vi "Display Module - Switch On and Off.vi"(0 "Image Refs":T1[](array[typedef]), 11 "IMAQ Display Refs":refnum<vi>[](array[refnum])) -> ()   [LabVIEW 2021]
uses:
  <vilib>/vision/Image Controls.llb/IMAQ Image.ctl
  <vilib>/Utility/miscctls.llb/LVPointTypeDef.ctl
panel:
  in  "Quit":bool
  # "Click on a display to change its state."
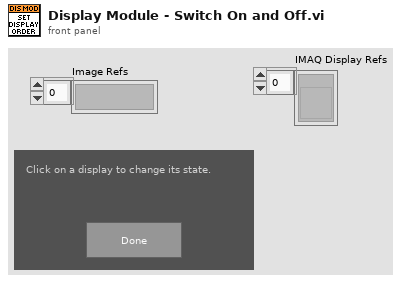
[diagram p1: front panel]
types:
  T1 = typedef "IMAQ Image.ctl" = refnum<image>
  T2 = enum16{"Always On", "Always Off", "Off While Running"}
  T3 = typedef "LVPointTypeDef.ctl" = cluster{"Horizontal":i16, "Vertical":i16}
  T4 = enum16{"User-specified Font", "Application Font", "System Font", "Dialog Font"}
  T5 = cluster{"Desired Font (Application)":enum16{"User-specified Font", "Application Font", "System Font", "Dialog Font"}, "[User-specified Font]":cluster{"Font Name":string, "Size":i16, "Strikeout?":bool, "Italic?":bool, "Underline?":bool, "Outline?":bool, "Shadow?":bool, "Bold?":bool, "Rotation Angle":dbl}, "Horizontal Alignment":i16, "Vertical Alignment":i16}
  T6 = cluster{"Font Name":string, "Size":i16, "Strikeout?":bool, "Italic?":bool, "Underline?":bool, "Outline?":bool, "Shadow?":bool, "Bold?":bool, "Rotation Angle":dbl}
  T7 = typedef "LVRectTypeDef.ctl" = cluster{"Left":i16, "Top":i16, "Right":i16, "Bottom":i16}
  T8 = typedef "LVBoundsTypeDef.ctl" = cluster{"Width":u32, "Height":u32}
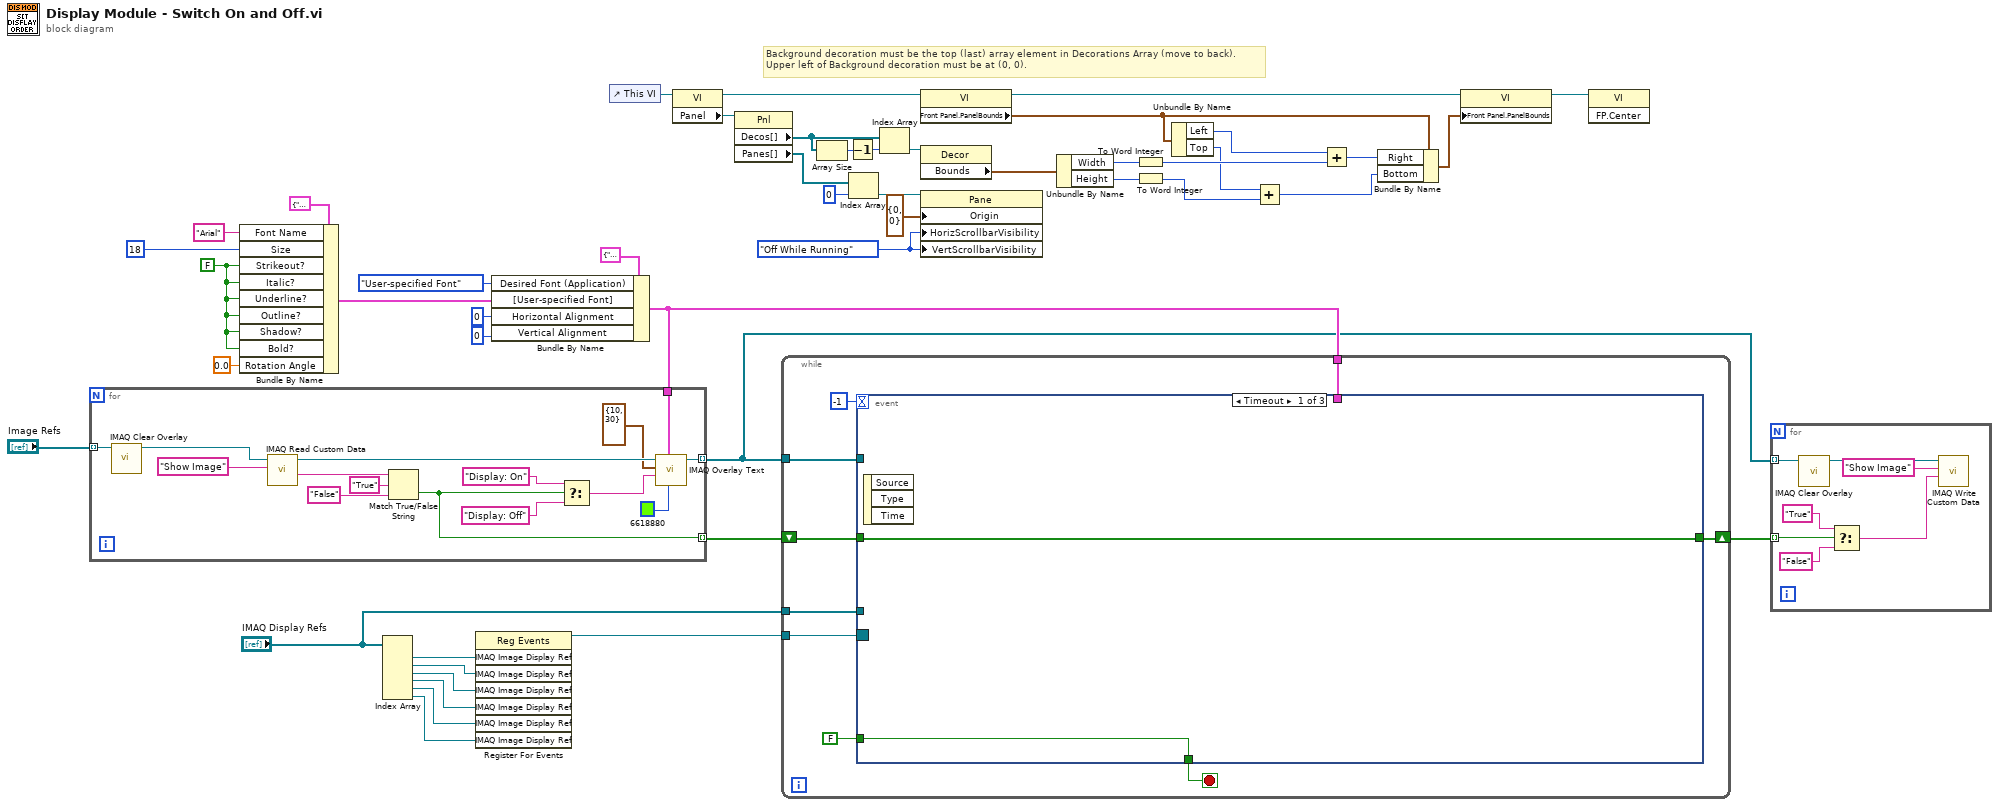
[diagram p0: block diagram]
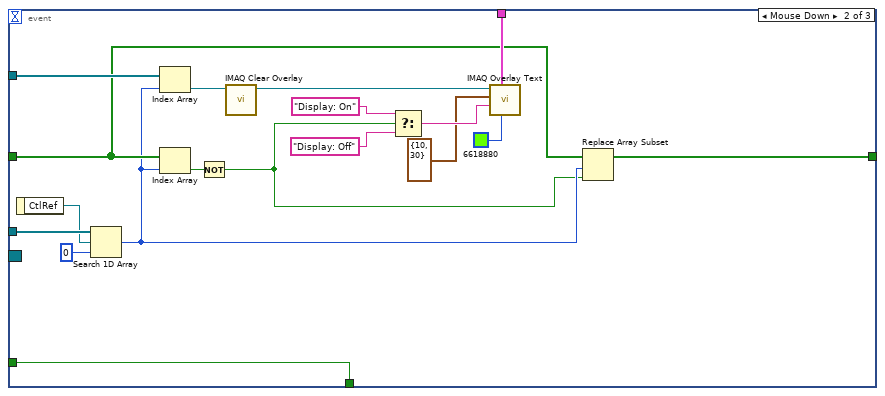
[diagram p2: hidden frame]
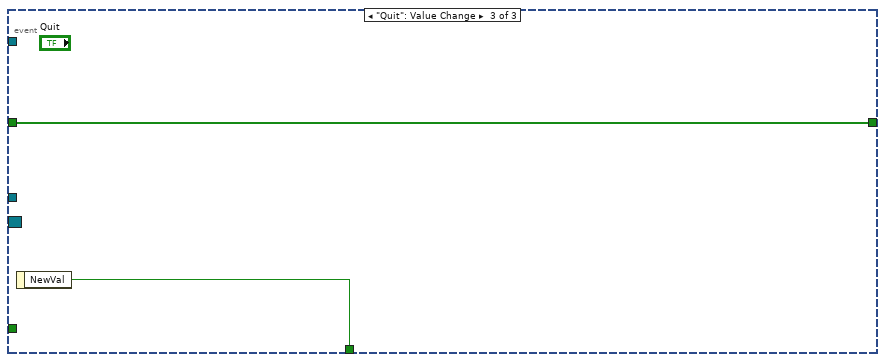
[diagram p3: hidden frame]
diagram:
  w15 = T2."Off While Running" ("Vertical Scrollbar Visibility")
  w38 = FALSE ("Strikeout?")
  # "Background decoration must be the top (last) array element in Decorations Array (move to back).\nUpper left of Background decoration must be at (0, 0)."
  n1 = Bundle By Name(cluster=T6 {"Font Name"="", "Size"=0, "Strikeout?"=FALSE, "Italic?"=FALSE, "Underline?"=FALSE, "Outline?"=FALSE, "Shadow?"=FALSE, "Bold?"=FALSE, "Rotation Angle"=0.0} ("[User-specified Font]"), "Font Name"="Arial", "Size"=i16 18, "Strikeout?"=w38, "Italic?"=w38, "Underline?"=w38, "Outline?"=w38, "Shadow?"=w38, "Bold?"=w38, "Rotation Angle"=0.0) -> (w40:T6)
  n2 = Index Array(array="IMAQ Display Refs") -> (element #1=w33:refnum<vi>, element #2=w37:refnum<vi>, element #3=w34:refnum<vi>, element #4=w35:refnum<vi>, element #5=w36:refnum<vi>, element #6=w31:refnum<vi>)  [unwired: 6 in]
  n3 = register-events(w33, w37, w34, w35, w36, w31) -> (reference out=w32:refnum<event-registration>)  [unwired: 2 in, 1 out]
  n4 = Bundle By Name(cluster=T5 {"Desired Font (Application)"=enum."Application Font", "[User-specified Font]"={"Font Name"="", "Size"=12, "Strikeout?"=FALSE, "Italic?"=FALSE, "Underline?"=FALSE, "Outline?"=FALSE, "Shadow?"=FALSE, "Bold?"=FALSE, "Rotation Angle"=0.0}, "Horizontal Alignment"=0, "Vertical Alignment"=0} ("Font, Size & Style"), "Desired Font (Application)"=T4."User-specified Font", "[User-specified Font]"=w40, "Horizontal Alignment"=i16 0, "Vertical Alignment"=i16 0) -> (w28:T5)
  n5 = for {
    tunnel: "Image Refs" -> [w52] mode=indexing
    tunnel: w28 -> [w53]
    tunnel: [w50] -> w27 mode=indexing
    tunnel: [w49] -> w30 mode=indexing
    n6 = call "IMAQ Clear Overlay"("Image"=w52) -> ("Image Out"=w51:T1)  [unwired: 9 in, 1 out]
    n7 = call "IMAQ Read Custom Data"("Key"="Show Image", "Image"=w51) -> ("Custom Data Out"=w63:string, "Image (duplicate)"=w59:T1)  [unwired: 7 in, 1 out]
    n8 = Match True/False String(2:"False" ("false string"), 3:"True" ("true string"), 4:w63) -> (0:w49:bool)  [unwired: 1 out]
    n9 = Select(t="Display: On" ("false string"), s=w49, f="Display: Off" ("false string")) -> (s? t:f=w55:string)
    n10 = call "IMAQ Overlay Text"("Text Color (black)"=u32 6618880, "Font, Size & Style"=w53, "String"=w55, "Origin"=cluster{"X":i32, "Y":i32} {"X"=10, "Y"=30}, "Image"=w59) -> ("Image Out"=w50:T1)  [unwired: 5 in, 1 out]
  }
  n11 = control-ref of="This VI"() -> (w8:refnum<vi>)
  n12 = property class="VI"(reference=w8) -> (reference out=w16:refnum<vi>, "Panel"=w9:refnum<vi>)  [unwired: 1 in, 1 out]
  n13 = property class="Pnl"(reference=w9) -> ("Decos[]"=w7:refnum<vi>[], "Panes[]"=w12:refnum<vi>[])  [unwired: 1 in, 2 out]
  n14 = while {
    tunnel: w32 -> [w69]
    shift-right: [w64] -> w26
    shift-left: w30 -> [w67]
    tunnel: "IMAQ Display Refs" -> [w66]
    tunnel: w28 -> [w65]
    tunnel: w27 -> [w68]
    stop <- w72 stop-if-true
    n15 = event shown="[0] Timeout" {
      selector: w69 -> [_ _ _]
      dyn-events: _ -> [_ _ _]
      timeout: -1 -> [_ _ _]
      tunnel: [w73 w92 w94] -> w72
      tunnel: FALSE -> [w73 w92 _]
      tunnel: w68 -> [_ w81 _]
      tunnel: w67 -> [w74 w78 w93]
      tunnel: w66 -> [_ w91 _]
      tunnel: w65 -> [_ w82 _]
      tunnel: [w74 w77 w93] -> w64
      event Timeout {
        n16 = event-data() -> ()  [unwired: 1 in, 3 out]
      }
      event Mouse Down {
        n17 = event-data() -> ("CtlRef"=w90:refnum<vi>)  [unwired: 1 in]
        n18 = Search 1D Array(1D array=w91, element=w90, start index (0)=0) -> (index of element=w76:i32)
        n19 = Index Array(array=w81, index=w76) -> (element=w80:T1)
        n20 = Index Array(array=w78, index=w76) -> (element=w88:bool)
        n21 = Not(x=w88) -> (.not. x?=w75:bool)
        n22 = call "IMAQ Clear Overlay"("Image"=w80) -> ("Image Out"=w79:T1)  [unwired: 9 in, 1 out]
        n23 = Select(t="Display: On" ("false string"), s=w75, f="Display: Off" ("false string")) -> (s? t:f=w84:string)
        n24 = call "IMAQ Overlay Text"("Text Color (black)"=u32 6618880, "Font, Size & Style"=w82, "String"=w84, "Origin"=cluster{"X":i32, "Y":i32} {"X"=10, "Y"=30}, "Image"=w79) -> ()  [unwired: 5 in, 2 out]
        n25 = Replace Array Subset(array=w78, new element=w75, index=w76) -> (w77:bool[])
      }
      event "Quit": Value Change {
        n26 = event-data() -> ("NewVal"=w94:bool)  [unwired: 1 in]
      }
    }
  }
  n27 = Array Size(array=w7) -> (size(s)=w5:i32)
  n28 = Decrement(x=w5) -> (x-1=w6:i32)
  n29 = Index Array(array=w12, index=0) -> (element=w11:refnum<vi>)
  n30 = Index Array(array=w7, index=w6) -> (element=w14:refnum<vi>)
  n31 = property class="VI"(reference=w16) -> (reference out=w18:refnum<vi>, "Front Panel.PanelBounds"=w19:T7)  [unwired: 1 in, 1 out]
  n32 = property class="Decor"(reference=w14) -> ("Bounds"=w17:T8)  [unwired: 1 in, 2 out]
  n33 = property class="Pane"(reference=w11, "Origin"=T3 {"Horizontal"=0, "Vertical"=0}, "HorizScrollbarVisibility"=w15, "VertScrollbarVisibility"=w15) -> ()  [unwired: 1 in, 2 out]
  n34 = Unbundle By Name(w17) -> ("Width"=w22:u32, "Height"=w25:u32)
  n35 = To Word Integer(number=w22) -> (16bit integer=w24:i16)
  n36 = To Word Integer(number=w25) -> (16bit integer=w3:i16)
  n37 = Unbundle By Name(w19) -> ("Left"=w21:i16, "Top"=w4:i16)
  n38 = Add(x=w4, y=w3) -> (x+y=w2:i16)
  n39 = Add(x=w21, y=w24) -> (x+y=w23:i16)
  n40 = Bundle By Name(cluster=w19, "Right"=w23, "Bottom"=w2) -> (w20:T7)
  n41 = property class="VI"(reference=w18, "Front Panel.PanelBounds"=w20) -> (reference out=w1:refnum<vi>)  [unwired: 1 in, 1 out]
  n42 = invoke class="VI" method="FP.Center"(reference=w1) -> ()  [unwired: 2 in, 3 out]
  n43 = for {
    tunnel: w27 -> [w98] mode=indexing
    tunnel: w26 -> [w101] mode=indexing
    n44 = call "IMAQ Clear Overlay"("Image"=w98) -> ("Image Out"=w97:T1)  [unwired: 9 in, 1 out]
    n45 = Select(t="True", s=w101, f="False") -> (s? t:f=w95:string)
    n46 = call "IMAQ Write Custom Data"("Custom Data In"=w95, "Key"="Show Image", "Image"=w97) -> ()  [unwired: 7 in, 2 out]
  }
